vi "Place_Middle_Gear_Auto.vi"(0 "Encoder_In":dbl=-835.5930827386422, 1 "Yaw_In":dbl=131.76181033780495, 2 "DBParams":T2={"MiddleAutoDist (in)"=-40.0, "SideAutoDist (in)"=-15.0, "AutoSpeed"=0.6, "RailCenterOffset (in)"=0.0, "RedAllianceRPM"=3700.0, "BlueAllianceRPM"=3400.0, "BaselineRPM"=0.0}, 3 "Place_Finished?":bool, 4 "Alliance":T1, 6 "Turning_Angle":dbl=30.0, 7 "Start?":bool, 11 "AutoMode":T3=enum."GearLeft") -> (10 "ShooterSpeedOutput (rpm)":dbl, 12 "RunFeeder":bool, 13 "Turning_Speed":dbl, 14 "Drive_PID_Enable":bool, 15 "Place_Gear?":bool, 17 "Current_State":T4, 18 "Desired_Yaw":dbl=116.89864520342934, 19 "Drive_Speed":dbl)   [LabVIEW 2016]
uses:
  TypeDefs/Auto_PlaceMiddleGearState_Type.ctl
  TypeDefs/AutoMode_Type.ctl
  TypeDefs/DB/dbParams_Type.ctl
  <vilib>/Rock Robotics/WPI/DriverStation/WPI_DriverStationAllianceInfo.ctl
  ArgosLib/Signal Processing/TypeDefs/EdgeDetector_Type.ctl
  ArgosLib/ArgosLib.lvlib
panel:
  in  "PlaceGearBrakeSpeed":dbl=0.05 format="%#_13g"
  in  "SidePegSubtractDist":dbl=15.0 format="%#_13g"
  in  "ShootTime (ms)":u32=4000
  in  "SpinUpTime (ms)":u32=1000
  in  "turnSpeed":dbl=0.4 format="%#_13g"
  in  "Forward_Drive_Distance":dbl=20.0
  in  "Forward_Drive_Speed":dbl=-0.5 format="%#_13g"
  # "Blue = 3400\nRed = 3700"
  # "Deprecated"
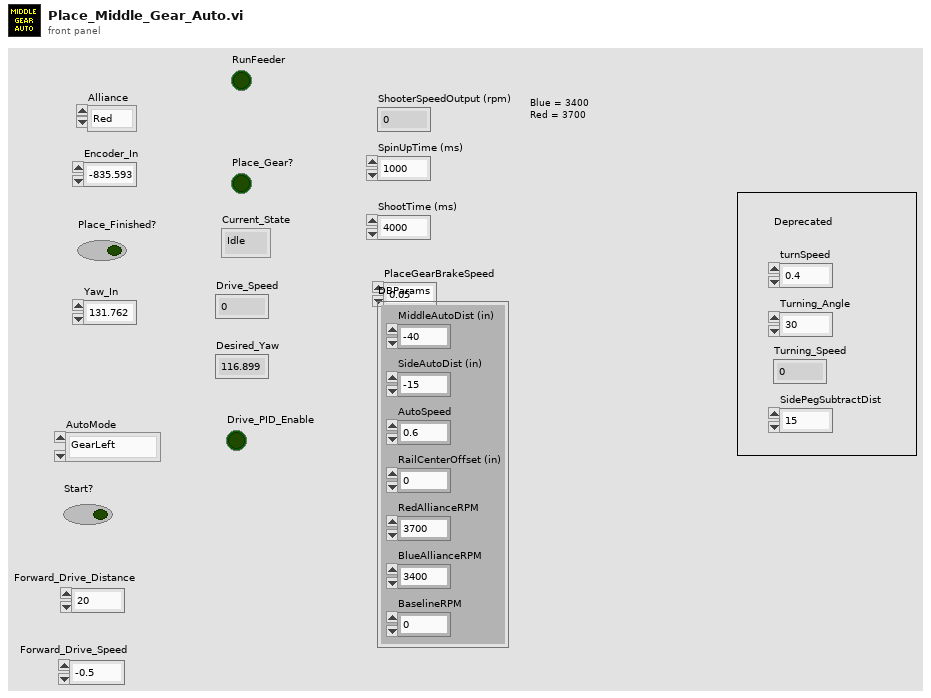
[diagram p1: front panel]
types:
  T1 = typedef "WPI_DriverStationAllianceInfo.ctl" = enum16{"Red", "Blue", "Invalid"}
  T2 = typedef "dbParams_Type.ctl" = cluster{"MiddleAutoDist (in)":dbl, "SideAutoDist (in)":dbl, "AutoSpeed":dbl, "RailCenterOffset (in)":dbl, "RedAllianceRPM":dbl, "BlueAllianceRPM":dbl, "BaselineRPM":dbl}
  T3 = typedef "AutoMode_Type.ctl" = enum16{"GearRight", "GearMiddle", "GearLeft", "Shoot&GearMiddle", "BaselineOnly", "Shoot&Baseline"}
  T4 = typedef "Auto_PlaceMiddleGearState_Type.ctl" = enum16{"Idle", "Drive", "Place_Gear", "Drive_Backwards", "Continue_Forward", "Turn", "SpinUp", "Shoot", "Stop"}
  T5 = typedef "EdgeDetector_Type.ctl" = enum16{"RisingEdge", "FallingEdge", "Both"}
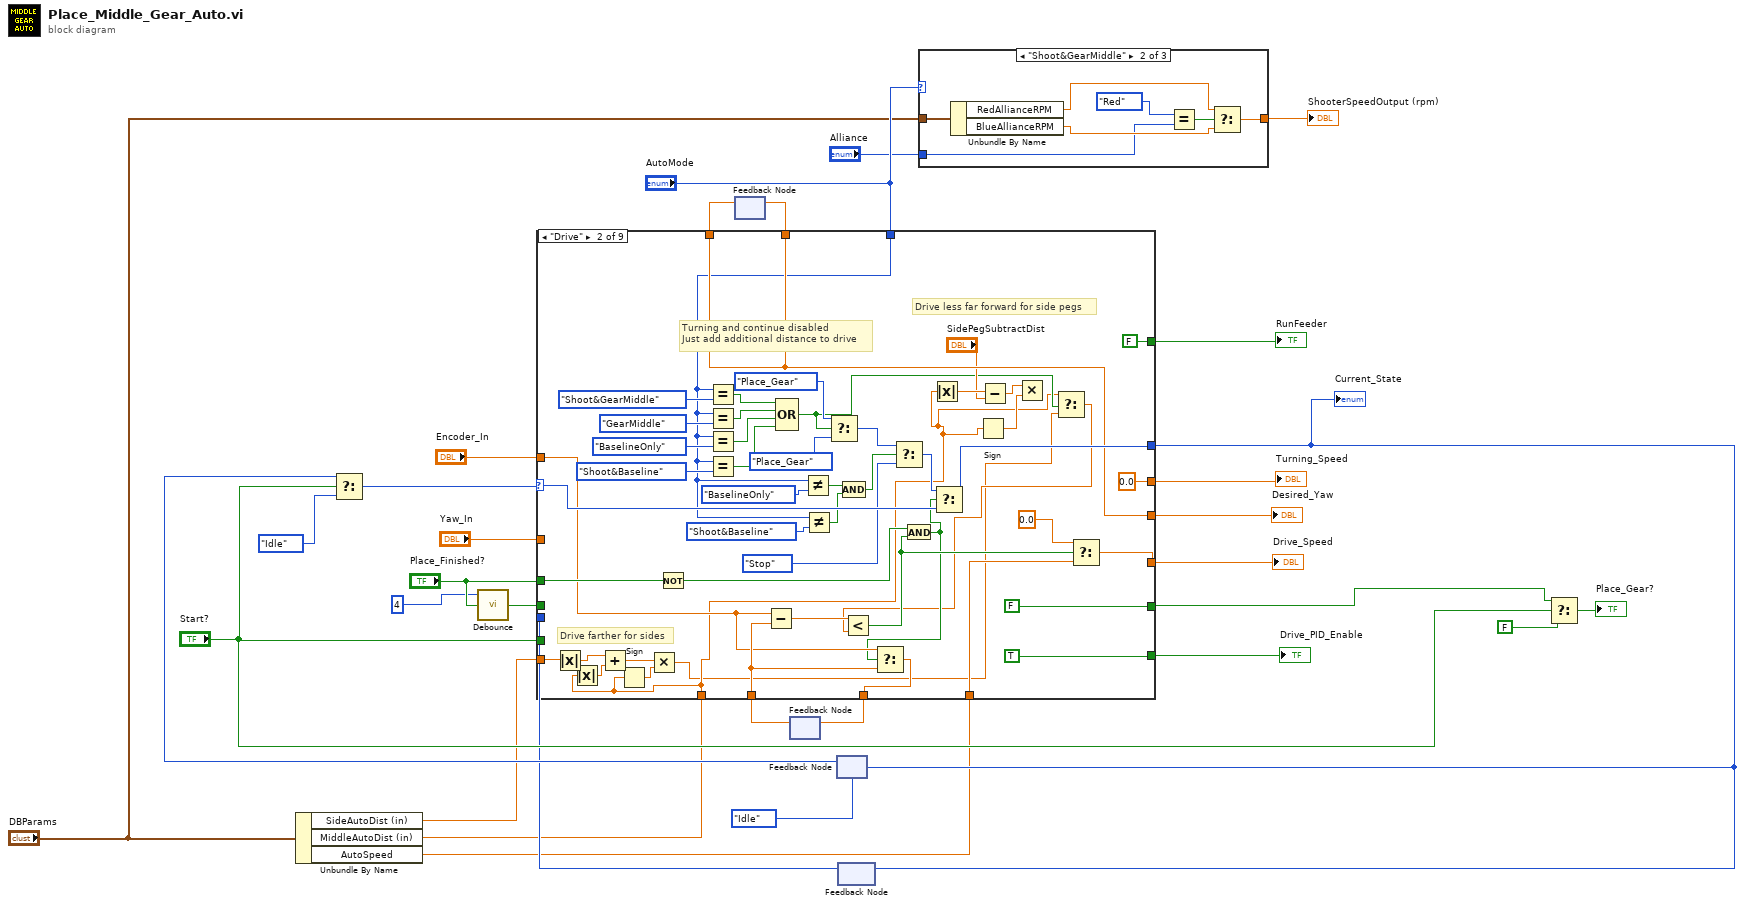
[diagram p0: block diagram]
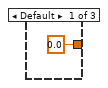
[diagram p2: hidden frame]
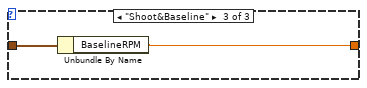
[diagram p3: hidden frame]
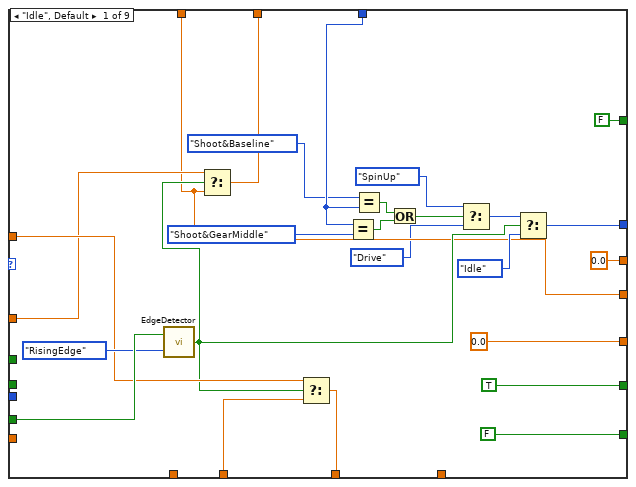
[diagram p4: hidden frame]
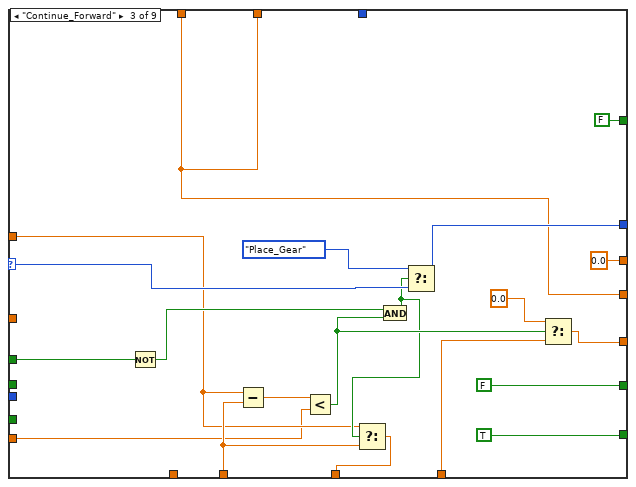
[diagram p5: hidden frame]
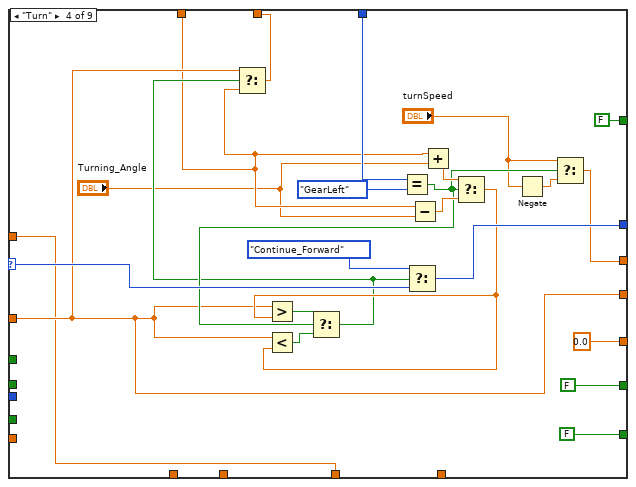
[diagram p6: hidden frame]
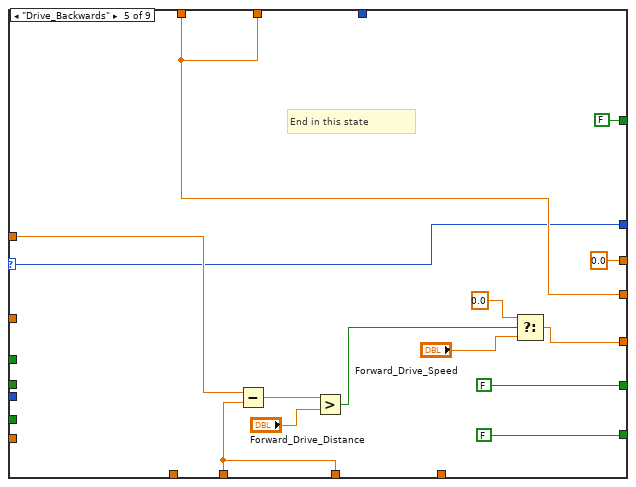
[diagram p7: hidden frame]
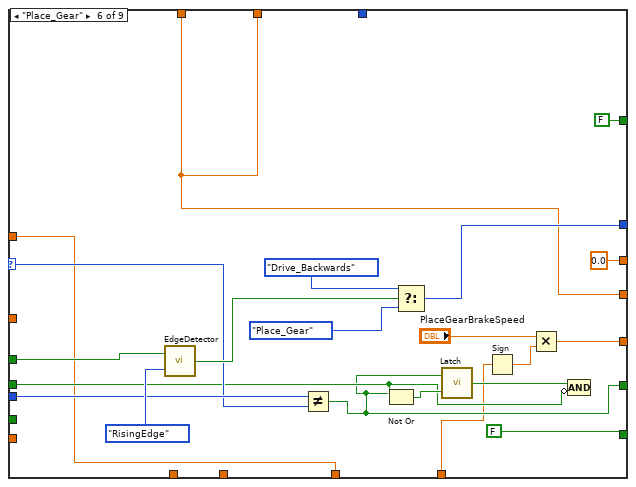
[diagram p8: hidden frame]
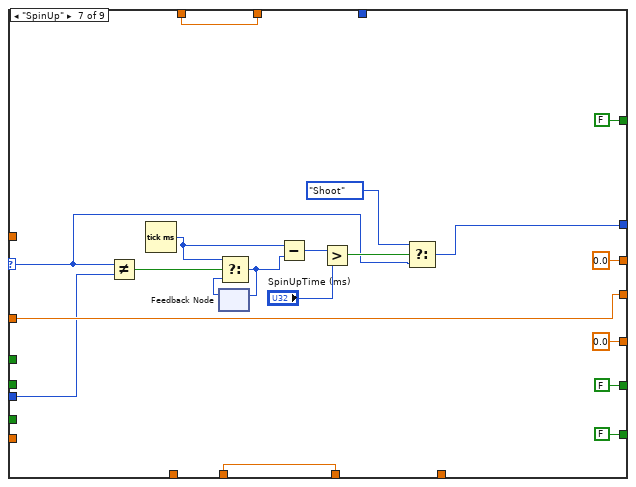
[diagram p9: hidden frame]
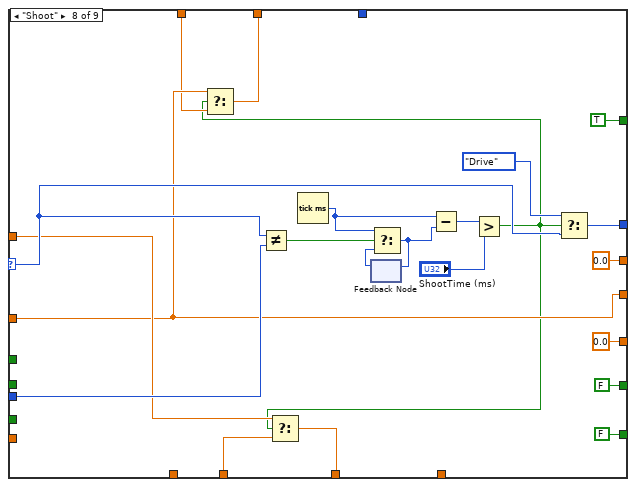
[diagram p10: hidden frame]
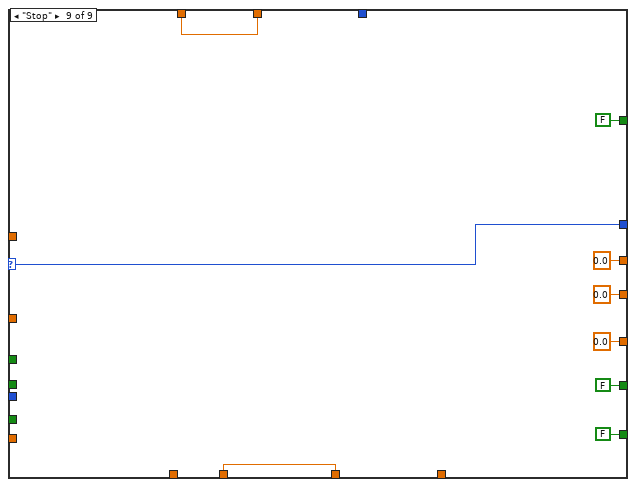
[diagram p11: hidden frame]
diagram:
  n1 = Unbundle By Name("DBParams") -> ("SideAutoDist (in)"=w5:dbl, "MiddleAutoDist (in)"=w6:dbl, "AutoSpeed"=w7:dbl)
  n2 = call "Debounce.vi"("Input"="Place_Finished?", "Num samples"=4) -> ("Output"=w10:bool)  [unwired: 1 in]
  n3 = feedback #1() -> (w24:dbl)  [unwired: 1 in]
  n4 = feedback #2() -> (w26:dbl)  [unwired: 1 in]
  n5 = feedback #3(Auto_PlaceMiddleGearState_Type."Idle") -> (w16:T4)
  n6 = Select(t=w16, s="Start?", f=Auto_PlaceMiddleGearState_Type."Idle") -> (s? t:f=w20:T4)
  n7 = feedback #4() -> (w13:T4)  [unwired: 1 in]
  n8 = case shown="\"Drive\"" w20 {
    selector: w20 -> [_ w94 w113 w148 w153 w177 w189 w218 w234]
    tunnel: "Encoder_In" -> [w50 w88 w110 w132 w163 w170 _ w210 _]
    tunnel: "Start?" -> [w56 _ _ _ _ _ _ _ _]
    tunnel: [w53 w105 w125 w149 w153 w184 w187 w219 w234] -> w14
    tunnel: [TRUE FALSE FALSE FALSE FALSE w172 FALSE FALSE FALSE] -> w15
    tunnel: [0.0 ("Drive_Speed") w101 w120 0.0 ("Drive_Speed") w159 w167 0.0 ("Drive_Speed") 0.0 ("Drive_Speed") 0.0 ("Drive_Speed")] -> w29
    tunnel: "Place_Finished?" -> [_ w98 w117 _ _ w176 _ _ _]
    tunnel: "Yaw_In" -> [w47 _ _ w134 _ _ w203 w209 _]
    tunnel: [w49 w86 w109 w132 w161 w170 w198 w212 w228] -> w27
    tunnel: w26 -> [w48 w89 w111 _ w161 _ w198 w211 w228]
    tunnel: [w45 w103 w122 w135 w155 w180 w199 w207 w227] -> w25
    tunnel: w24 -> [w44 w103 w122 w129 w155 w180 w199 w208 w227]
    tunnel: [w44 w103 w122 w134 w155 w180 w203 w209 0.0 ("Yaw_In")] -> w23
    tunnel: [FALSE TRUE TRUE FALSE FALSE FALSE FALSE FALSE FALSE] -> w22
    tunnel: w13 -> [_ _ _ _ _ w178 w197 w217 _]
    tunnel: w10 -> [_ _ _ _ _ w173 _ _ _]
    tunnel: "AutoMode" -> [w33 w61 _ w142 _ _ _ _ _]
    tunnel: w7 -> [_ w96 w115 _ _ w168 _ _ _]
    tunnel: w6 -> [_ w69 _ _ _ _ _ _ _]
    tunnel: [0.0 ("f") 0.0 ("f") 0.0 ("f") w140 0.0 ("f") 0.0 ("f") 0.0 ("f") 0.0 ("f") 0.0 ("f")] -> w9
    tunnel: [FALSE FALSE FALSE FALSE FALSE FALSE FALSE TRUE FALSE] -> w8
    tunnel: w5 -> [_ w72 w107 _ _ _ _ _ _]
    frame "Idle", Default {
      n9 = call "EdgeDetector.vi"("DetectorType"=EdgeDetector_Type."RisingEdge", "Input"=w56) -> ("Edge"=w46:bool)
      n10 = Select(t=w47, s=w46, f=w44) -> (s? t:f=w45:dbl)
      n11 = Select(t=w50, s=w46, f=w48) -> (s? t:f=w49:dbl)
      n12 = Equal?(x=w33, y=AutoMode_Type."Shoot&GearMiddle") -> (x = y?=w41:bool)
      n13 = Equal?(x=AutoMode_Type."Shoot&Baseline", y=w33) -> (x = y?=w34:bool)
      n14 = Or(x=w34, y=w41) -> (x .or. y?=w35:bool)
      n15 = Select(t=Auto_PlaceMiddleGearState_Type."SpinUp", s=w35, f=Auto_PlaceMiddleGearState_Type."Drive") -> (s? t:f=w40:T4)
      n16 = Select(t=w40, s=w46, f=Auto_PlaceMiddleGearState_Type."Idle") -> (s? t:f=w53:T4)
    }
    frame "Drive" {
      # "Drive farther for sides"
      # "Turning and continue disabled\nJust add additional distance to drive"
      # "Drive less far forward for side pegs"
      n17 = Absolute Value(x=w72) -> (abs(x)=w71:dbl)
      n18 = Absolute Value(x=w69) -> (abs(x)=w70:dbl)
      n19 = Add(x=w71, y=w70) -> (x+y=w67:dbl)
      n20 = Sign(1:w69) -> (0:w68:dbl)
      n21 = Multiply(x=w67, y=w68) -> (x*y=w66:dbl)
      n22 = Not(x=w98) -> (.not. x?=w97:bool)
      n23 = Equal?(x=w61, y=AutoMode_Type."Shoot&GearMiddle") -> (x = y?=w78:bool)
      n24 = Equal?(x=w61, y=AutoMode_Type."GearMiddle") -> (x = y?=w77:bool)
      n25 = Equal?(x=w61, y=AutoMode_Type."BaselineOnly") -> (x = y?=w64:bool)
      n26 = Equal?(x=w61, y=AutoMode_Type."Shoot&Baseline") -> (x = y?=w62:bool)
      n27 = Subtract(x=w88, y=w89) -> (x-y=w104:dbl)
      n28 = Compound Arithmetic op=OR(w78, w77, w64, w62) -> (w76:bool)
      n29 = Not Equal?(x=w61, y=AutoMode_Type."BaselineOnly") -> (x != y?=w59:bool)
      n30 = Not Equal?(x=w61, y=AutoMode_Type."Shoot&Baseline") -> (x != y?=w58:bool)
      n31 = Select(t=Auto_PlaceMiddleGearState_Type."Place_Gear", s=w76, f=Auto_PlaceMiddleGearState_Type."Place_Gear") -> (s? t:f=w92:T4)
      n32 = Compound Arithmetic op=AND(w59, w58) -> (w57:bool)
      n33 = Select(t=w92, s=w57, f=Auto_PlaceMiddleGearState_Type."Stop") -> (s? t:f=w75:T4)
      n34 = Absolute Value(x=w69) -> (abs(x)=w84:dbl)
      n35 = Sign(1:w69) -> (0:w81:dbl)
      n36 = Subtract(x=w84, y="SidePegSubtractDist") -> (x-y=w82:dbl)
      n37 = Multiply(x=w82, y=w81) -> ()  [unwired: 1 out]
      n38 = Select(t=w69, s=w76, f=w66) -> (s? t:f=w80:dbl)
      n39 = Less?(x=w104, y=w80) -> (x < y?=w99:bool)
      n40 = And(x=w97, y=w99) -> (x .and. y?=w87:bool)
      n41 = Select(t=w88, s=w87, f=w89) -> (s? t:f=w86:dbl)
      n42 = Select(t=w75, s=w87, f=w94) -> (s? t:f=w105:T4)
      n43 = Select(t=0.0, s=w99, f=w96) -> (s? t:f=w101:dbl)
    }
    frame "Continue_Forward" {
      n44 = Not(x=w117) -> (.not. x?=w116:bool)
      n45 = Subtract(x=w110, y=w111) -> (x-y=w123:dbl)
      n46 = Less?(x=w123, y=w107) -> (x < y?=w118:bool)
      n47 = And(x=w116, y=w118) -> (x .and. y?=w112:bool)
      n48 = Select(t=w110, s=w112, f=w111) -> (s? t:f=w109:dbl)
      n49 = Select(t=Auto_PlaceMiddleGearState_Type."Place_Gear", s=w112, f=w113) -> (s? t:f=w125:T4)
      n50 = Select(t=0.0, s=w118, f=w115) -> (s? t:f=w120:dbl)
    }
    frame "Turn" {
      n51 = Equal?(x=w142, y=AutoMode_Type."GearLeft") -> (x = y?=w138:bool)
      n52 = Subtract(x=w129, y="Turning_Angle") -> (x-y=w147:dbl)
      n53 = Add(x=w129, y="Turning_Angle") -> (x+y=w146:dbl)
      n54 = Select(t=w146, s=w138, f=w147) -> (s? t:f=w136:dbl)
      n55 = Greater?(x=w134, y=w136) -> (0:w139:bool)
      n56 = Less?(x=w134, y=w136) -> (x < y?=w137:bool)
      n57 = Select(t=w139, s=w138, f=w137) -> (s? t:f=w133:bool)
      n58 = Select(t=w134, s=w133, f=w129) -> (s? t:f=w135:dbl)
      n59 = Select(t=Auto_PlaceMiddleGearState_Type."Continue_Forward", s=w133, f=w148) -> (s? t:f=w149:T4)
      n60 = Negate(x="turnSpeed") -> (-x=w131:dbl)
      n61 = Select(t="turnSpeed", s=w138, f=w131) -> (s? t:f=w140:dbl)
    }
    frame "Drive_Backwards" {
      # "End in this state"
      n62 = Subtract(x=w163, y=w161) -> (x-y=w162:dbl)
      n63 = Greater?(x=w162, y="Forward_Drive_Distance") -> (0:w157:bool)
      n64 = Select(t=0.0, s=w157, f="Forward_Drive_Speed") -> (s? t:f=w159:dbl)
    }
    frame "Place_Gear" {
      n65 = call "EdgeDetector.vi"("DetectorType"=EdgeDetector_Type."RisingEdge", "Input"=w176) -> ("Edge"=w182:bool)
      n66 = Not Equal?(x=w178, y=w177) -> (x != y?=w172:bool)
      n67 = Not Or(1:w173, 2:w172) -> (0:w175:bool)
      n68 = Select(t=Auto_PlaceMiddleGearState_Type."Drive_Backwards", s=w182, f=Auto_PlaceMiddleGearState_Type."Place_Gear") -> (s? t:f=w184:T4)
      n69 = call "Latch.vi"("Reset"=w175, "Input"=w172) -> ("LatchOut"=w174:bool)
      n70 = Sign(1:w168) -> (0:w165:dbl)
      n71 = Multiply(x="PlaceGearBrakeSpeed", y=w165) -> (x*y=w167:dbl)
      n72 = Compound Arithmetic op=AND(w174, invert w173) -> ()  [unwired: 1 out]
    }
    frame "SpinUp" {
      n73 = Not Equal?(x=w189, y=w197) -> (x != y?=w196:bool)
      n74 = Tick Count (ms)() -> (millisecond timer value=w195:u32)
      n75 = feedback #5() -> (w193:u32)  [unwired: 1 in]
      n76 = Select(t=w195, s=w196, f=w193) -> (s? t:f=w194:u32)
      n77 = feedback-in #5(w194) -> ()
      n78 = Subtract(x=w195, y=w194) -> (x-y=w192:u32)
      n79 = Greater?(x=w192, y="SpinUpTime (ms)") -> (0:w190:bool)
      n80 = Select(t=Auto_PlaceMiddleGearState_Type."Shoot", s=w190, f=w189) -> (s? t:f=w187:T4)
    }
    frame "Shoot" {
      n81 = Not Equal?(x=w218, y=w217) -> (x != y?=w226:bool)
      n82 = Tick Count (ms)() -> (millisecond timer value=w225:u32)
      n83 = feedback #6() -> (w223:u32)  [unwired: 1 in]
      n84 = Select(t=w225, s=w226, f=w223) -> (s? t:f=w224:u32)
      n85 = feedback-in #6(w224) -> ()
      n86 = Subtract(x=w225, y=w224) -> (x-y=w222:u32)
      n87 = Greater?(x=w222, y="ShootTime (ms)") -> (0:w206:bool)
      n88 = Select(t=w209, s=w206, f=w208) -> (s? t:f=w207:dbl)
      n89 = Select(t=w210, s=w206, f=w211) -> (s? t:f=w212:dbl)
      n90 = Select(t=Auto_PlaceMiddleGearState_Type."Drive", s=w206, f=w218) -> (s? t:f=w219:T4)
    }
    frame "Stop" {
    }
  }
  "Current_State" <- w14
  "Desired_Yaw" <- w23
  "Drive_PID_Enable" <- w22
  "Drive_Speed" <- w29
  "Turning_Speed" <- w9
  "RunFeeder" <- w8
  n91 = feedback-in #1(w25) -> ()
  n92 = feedback-in #2(w27) -> ()
  n93 = feedback-in #3(w14) -> ()
  n94 = feedback-in #4(w14) -> ()
  n95 = case shown="\"Shoot&GearMiddle\"" "AutoMode" {
    tunnel: [0.0 ("f") w239 w244] -> w3
    tunnel: "DBParams" -> [_ w238 w245]
    tunnel: "Alliance" -> [_ w237 _]
    frame Default {
    }
    frame "Shoot&GearMiddle" {
      n96 = Unbundle By Name(w238) -> ("RedAllianceRPM"=w242:dbl, "BlueAllianceRPM"=w243:dbl)
      n97 = Equal?(x=WPI_DriverStationAllianceInfo."Red" ("Alliance"), y=w237) -> (x = y?=w241:bool)
      n98 = Select(t=w242, s=w241, f=w243) -> (s? t:f=w239:dbl)
    }
    frame "Shoot&Baseline" {
      n99 = Unbundle By Name(w245) -> ("BaselineRPM"=w244:dbl)
    }
  }
  "ShooterSpeedOutput (rpm)" <- w3
  n100 = Select(t=w15, s="Start?", f=FALSE) -> (s? t:f=→"Place_Gear?":bool)
